vi "RDC-water-generate_perm_param_to_share.vi"(11 "Stop Temp":dbl=40.0) -> (0 "used temp":dbl)   [LabVIEW 2020, in "RDC-Reflection_Data_Computation.lvlib"]
doc: "Formats the water model parameters per temperature, up to Stop Temp, into a text table on the panel."
uses:
  RDC-Reflection_Data_Computation.lvlib
  RDC-water-param.ctl
panel:
  out "Array":T1[](array[typedef]) {"tau" format="%#.9e"}
  out "String":string
  in  "Increment temp":dbl=5.0
  in  "Start temp":dbl=10.0
  out "unsigned 16bit integer":i32
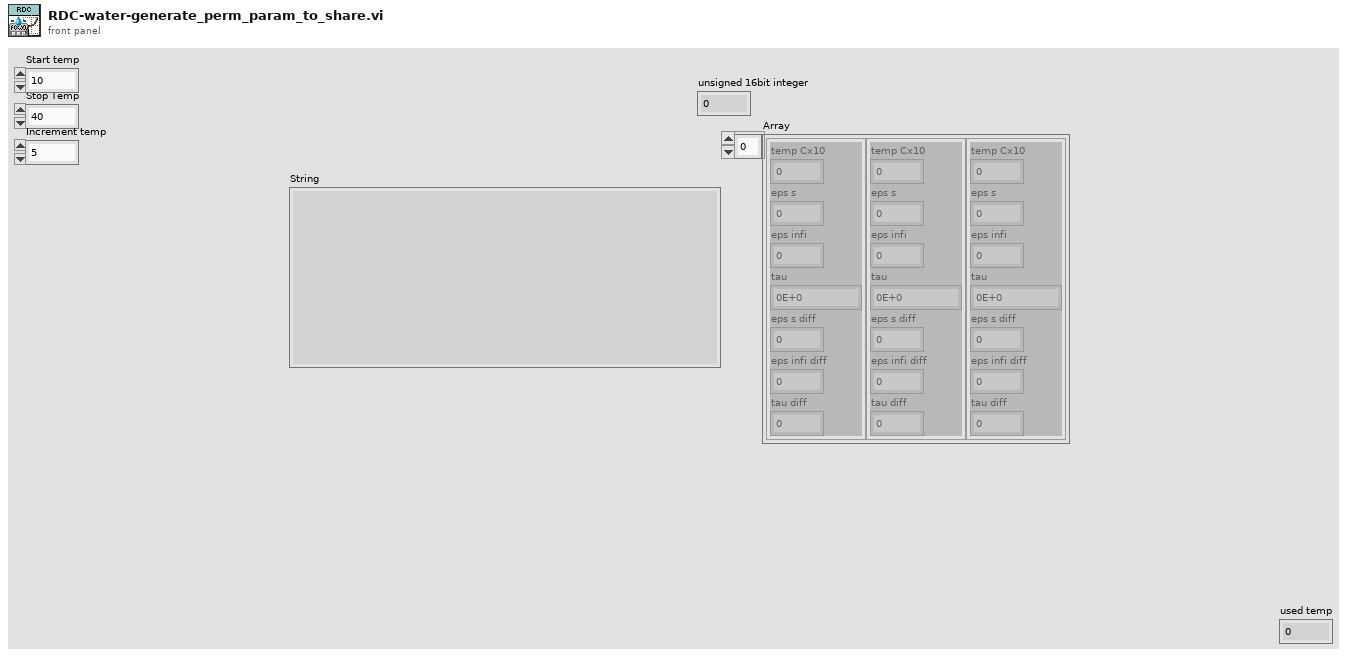
[diagram p1: front panel]
types:
  T1 = typedef "RDC-Reflection_Data_Computation.lvlib/RDC-water-param.ctl" = cluster{"temp Cx10":u16, "eps s":dbl, "eps infi":dbl, "tau":dbl, "eps s diff":dbl, "eps infi diff":dbl, "tau diff":dbl}
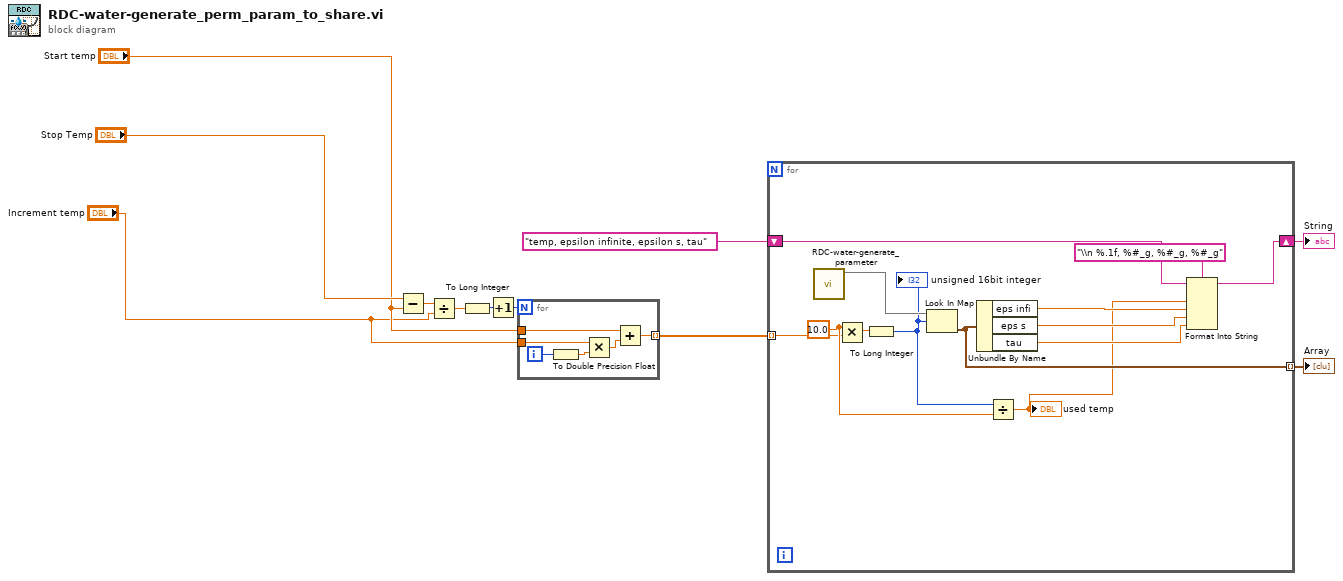
[diagram p0: block diagram]
diagram:
  n1 = Subtract(x="Stop Temp", y="Start temp") -> (x-y=w11:dbl)
  n2 = Divide(x=w11, y="Increment temp") -> (x/y=w10:dbl)
  n3 = To Long Integer(number=w10) -> (32bit integer=w9:i32)
  n4 = Increment(x=w9) -> (x+1=w8:i32)
  n5 = for {
    N: w8 -> [_]
    tunnel: "Start temp" -> [w15]
    tunnel: "Increment temp" -> [w14]
    tunnel: [w12] -> w4 mode=indexing
    i -> [w13]
    n6 = To Double Precision Float(number=w13) -> (double precision float=w17:dbl)
    n7 = Multiply(x=w14, y=w17) -> (x*y=w16:dbl)
    n8 = Add(x=w15, y=w16) -> (x+y=w12:dbl)
  }
  n9 = for {
    tunnel: w4 -> [w26] mode=indexing
    shift-right: [w25] -> w2
    shift-left: "temp, epsilon infinite, epsilon s, tau" -> [w24]
    tunnel: [w19] -> w1 mode=indexing
    w27 = 10.0 ("x")
    n10 = call "RDC-water-generate_parameter.vi"() -> ("parameter map"=w29:map{i32, T1})  [unwired: 11 in]
    n11 = Multiply(x=w27, y=w26) -> (x*y=w30:dbl)
    n12 = To Long Integer(number=w30) -> (32bit integer=w28:i32)
    "unsigned 16bit integer" <- w28
    n13 = Look In Map(map=w29, key=w28) -> (value=w19:T1)  [unwired: 1 in, 1 out]
    n14 = Unbundle By Name(w19) -> ("eps infi"=w22:dbl, "eps s"=w21:dbl, "tau"=w20:dbl)
    n15 = Divide(x=w28, y=w27) -> (x/y=w18:dbl)
    "used temp" <- w18
    n16 = Format Into String(format string="\\n %.1f, %#_g, %#_g, %#_g", initial string=w24, w18, w22, w21, w20) -> (resulting string=w25:string)  [unwired: 1 in, 1 out]
  }
  "String" <- w2
  "Array" <- w1
